vi "SetValueByItemTag.vi"(0 "VI Reference In":refnum<vi>, 2 "delimiter (>>)":string=">>", 5 "Control Path":string, 7 "Item Tag":string, 11 "Error In":errorcluster) -> (4 "VI Reference Out":refnum<vi>, 15 "Error Out":errorcluster)   [LabVIEW 2016, in "Drona.lvlib" / "ControlValue.lvlib" / "StimulusTree.lvlib"]
doc: "Sets value(signaling) for the tree control whose item tag is specified. \n\nThe input control name is given as a string , incase of path, use delimiters inbetween the path."
uses:
  StimulusTree.lvlib
  <vilib>/Utility/error.llb/Error Cluster From Error Code.vi
  <vilib>/ErrorRing/Error Ring.xnode
  Drona.lvlib
  Get/GetControlRef/GetControlRef.lvlib
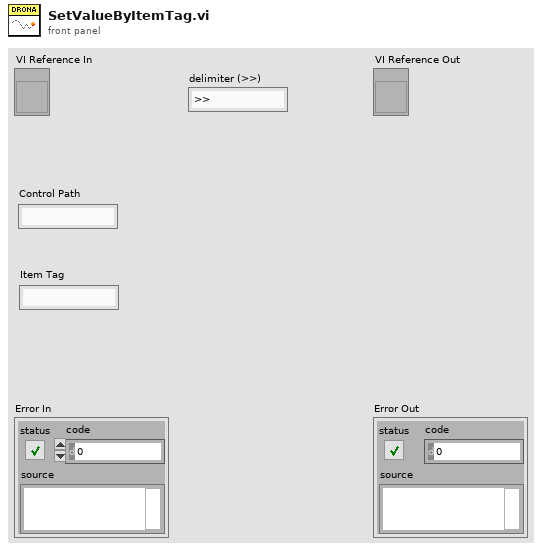
[diagram p1: front panel]
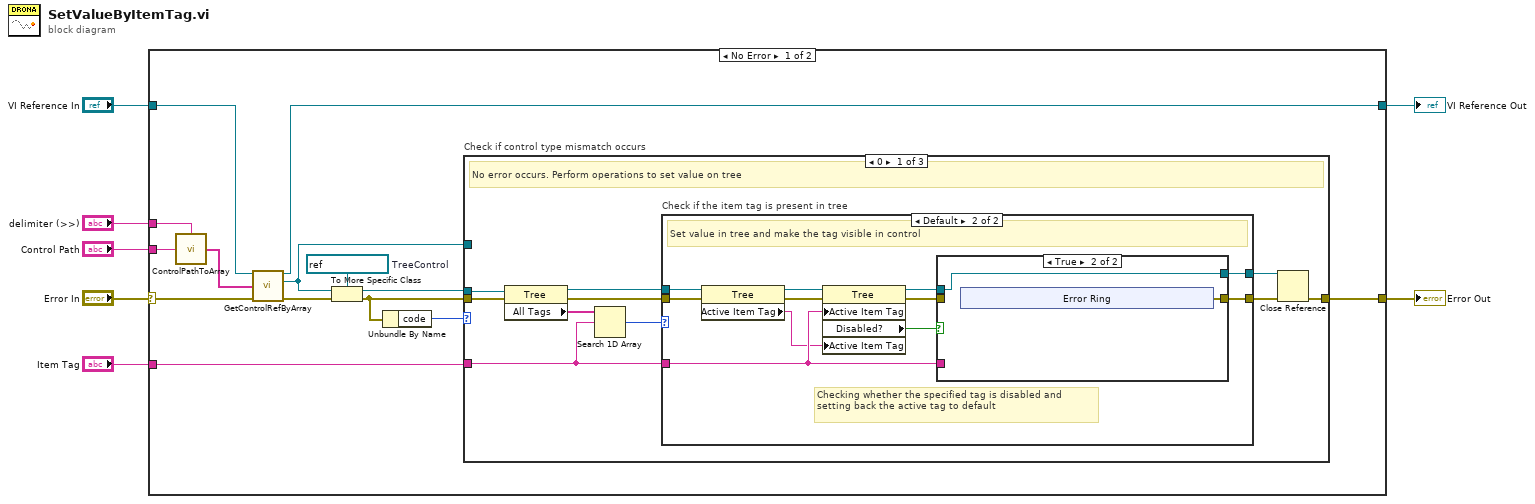
[diagram p0: block diagram]
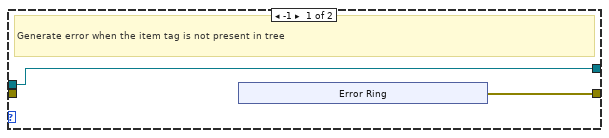
[diagram p2: hidden frame]
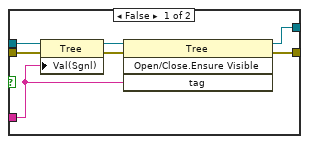
[diagram p3: hidden frame]
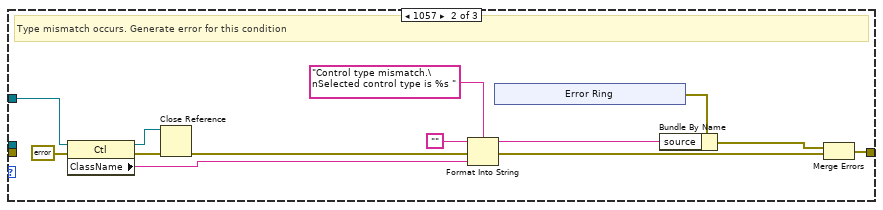
[diagram p4: hidden frame]
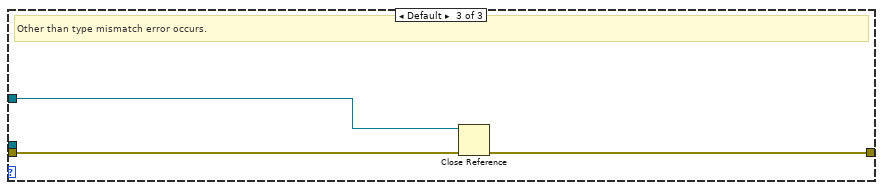
[diagram p5: hidden frame]
diagram:
  n1 = case shown="No Error" "Error In" {
    selector: "Error In" -> [w18 w86]
    tunnel: [w9 w86] -> w6
    tunnel: "VI Reference In" -> [w17 w85]
    tunnel: "Control Path" -> [w20 _]
    tunnel: [w14 w85] -> w3
    tunnel: "delimiter (>>)" -> [w19 _]
    tunnel: "Item Tag" -> [w10 _]
    frame No Error {
      w21 = refnum<vi> refnum  # TreeControl
      n2 = call "ControlPathToArray.vi"("Control Name"=w20, "delimiter (>>)"=w19) -> ("Control Path"=w16:string[])
      n3 = call "GetControlRefByArray.vi"("VI Reference In"=w17, "Control Path"=w16, "error In"=w18) -> ("VI Reference Out"=w14:refnum<vi>, "Ctl Refnum"=w11:refnum<vi>, "error out"=w15:errorcluster)  [unwired: 10 in]
      n4 = To More Specific Class(target class=w21, reference=w11, error in=w15) -> (specific class reference=w12:refnum<vi>, error out=w13:errorcluster)
      n5 = Unbundle By Name(w13) -> ("code"=w8:i32)
      n6 = case "Check if control type mismatch occurs" shown="0" w8 {
        tunnel: [w31 w66 w83] -> w9
        tunnel: w12 -> [w26 _ _]
        tunnel: w10 -> [w22 _ _]
        tunnel: w11 -> [_ w76 w82]
        tunnel: w13 -> [w30 _ w84]
        frame 0 {
          # "No error occurs. Perform operations to set value on tree"
          n7 = property class="Tree"(reference=w26, error in=w30) -> (reference out=w25:refnum<vi>, error out=w27:errorcluster, "All Tags"=w24:string[])
          n8 = Search 1D Array(1D array=w24, element=w22) -> (index of element=w23:i32)  [unwired: 1 in]
          n9 = case "Check if the item tag is present in tree" shown="Default" w23 {
            tunnel: [w32 w49] -> w29
            tunnel: [w33 w48] -> w28
            tunnel: w27 -> [_ w43]
            tunnel: w25 -> [w33 w41]
            tunnel: w22 -> [_ w45]
            frame -1 {
              # "Generate error when the item tag is not present in tree"
              n10 = xnode "Error Ring"() -> ("error out"=w32:errorcluster)
            }
            frame Default {
              # "Checking whether the specified tag is disabled and  setting back the active tag to default"
              # "Set value in tree and make the tag visible in control"
              n11 = property class="Tree"(reference=w41, error in=w43) -> (reference out=w40:refnum<vi>, error out=w42:errorcluster, "Active Item Tag"=w39:string)
              n12 = property class="Tree"(reference=w40, error in=w42, "Active Item Tag"=w45, "Active Item Tag"=w39) -> (reference out=w46:refnum<vi>, error out=w47:errorcluster, "Disabled?"=w44:bool)
              n13 = case shown="True" w44 {
                tunnel: w47 -> [w56 _]
                tunnel: w46 -> [w55 w58]
                tunnel: [w53 w57] -> w49
                tunnel: w45 -> [w51 _]
                tunnel: [w50 w58] -> w48
                frame False {
                  n14 = property class="Tree"(reference=w55, error in=w56, "Val(Sgnl)"=w51) -> (reference out=w52:refnum<vi>, error out=w54:errorcluster)
                  n15 = invoke class="Tree" method="Open/Close.Ensure Visible"(reference=w52, error in=w54, "tag"=w51) -> (reference out=w50:refnum<vi>, error out=w53:errorcluster)  [unwired: 1 in, 2 out]
                }
                frame True {
                  n16 = xnode "Error Ring"() -> ("error out"=w57:errorcluster)
                }
              }
            }
          }
          n17 = Close Reference(reference=w28, error in (no error)=w29) -> (error out=w31:errorcluster)
        }
        frame 1057 {
          # "Type mismatch occurs. Generate error for this condition"
          n18 = property class="Ctl"(reference=w76, error in=errorcluster {"status"=FALSE, "code"=0, "source"=""} ("error out")) -> (reference out=w64:refnum<vi>, error out=w75:errorcluster, "ClassName"=w72:string)
          n19 = Close Reference(reference=w64, error in (no error)=w75) -> (error out=w65:errorcluster)
          n20 = Format Into String(format string="Control type mismatch.\nSelected control type is %s ", initial string="", error in=w65, w72) -> (resulting string=w69:string, error out=w67:errorcluster)
          n21 = xnode "Error Ring"() -> ("error out"=w70:errorcluster)
          n22 = Bundle By Name(cluster=w70, "source"=w69) -> (w68:errorcluster)
          n23 = Merge Errors(w68, w67) -> (w66:errorcluster)
        }
        frame Default {
          # "Other than type mismatch error occurs."
          n24 = Close Reference(reference=w82, error in (no error)=w84) -> (error out=w83:errorcluster)
        }
      }
    }
    frame Error {
    }
  }
  "Error Out" <- w6
  "VI Reference Out" <- w3
